vi "Create.vi"(7 "Direction":T1, 8 "error in (no error)":errorcluster, 9 "Custom Config Data":u8[](array[numeric]), 10 "Name":string, 11 "CIFTag in":refnum<class "CIF_Iceoryx_Chn_String.lvclass">) -> (0 "error out":errorcluster, 3 "CIFTag out":refnum<class "CIF_Iceoryx_Chn_String.lvclass">)   [LabVIEW 2021, in "CIF_Iceoryx_Chn_String.lvclass"]
uses:
  CIF_Iceoryx_Chn_String.lvclass
  D:/dev/Packages/CIF_Channels_Core/src/Iceorxy_Channels/CIF_Iceoryx_BB/CIF_Iceoryx_BB.lvclass
  D:/dev/Packages/CIF_Channels_Core/src/CIFChannels/CIFChannels.lvclass
  ChannelCommon/typedef/Direction.ctl
  <vilib>/CIF Foundation/CIF Iceoryx/typedef/Topic Full Names.ctl
  ChannelCommon/typedef/Disconnect Behavior.ctl
  ChannelCommon/typedef/Channel Pattern.ctl
  CIF_Iceoryx_BB/CIF_Iceoryx_BB.lvclass/CIF_Iceoryx_BB.ctl
  ChannelCommon/typedef/Channel State.ctl
  CIFChannels/CIFChannels.lvclass/CIFChannels.ctl
  623fbe6a-c577-42e6-8857-c9eb486a6fdc.vi
  CIF_Iceoryx_BB/Accessors/Write Writer Reference.vi
  CIF_Iceoryx_BB/Accessors/Read Blackboard Reference.vi
  CIF_Iceoryx_BB/Accessors/Write Data Configuration.vi
  CIFChannels/Accessors/Write Pattern.vi
  CIFChannels/Accessors/Write Channel State.vi
  <vilib>/CIF Foundation/CIF Iceoryx/SubVIs/Get Path.vi
  <vilib>/CIF Foundation/CIF Iceoryx/SubVIs/Convert Error.vi
  623fbe6a-c577-42e6-8857-c9eb486a6fdc.vi/3bd89bd1-b605-4b55-aa60-227046f12b11.vi
  <vilib>/CIF Foundation/CIF Iceoryx/SubVIs/Add Error.vi
  <vilib>/CIF Foundation/CIF Iceoryx/Refnum/BB from Refnum.vi
  <vilib>/CIF Foundation/CIF Iceoryx/Refnum/BB Writer to Refnum.vi
  <vilib>/Utility/error.llb/Trim Whitespace.vi
  <vilib>/CIF Foundation/CIF Iceoryx/SubVIs/Add Error Core.vi
  <vilib>/CIF Foundation/CIF Utilities/DataTypes/Utilities/Get Element Info of Variant.vi
  <vilib>/CIF Foundation/CIF Iceoryx/SubVIs/Get Type String.vi
  <vilib>/CIF Foundation/CIF Utilities/DataTypes/Utilities/Get JSON Descriptor of Variant.vi
  <vilib>/CIF Foundation/CIF Iceoryx/SubVIs/Convert Error Core.vi
  CIFChannels/CIFChannels.lvclass
  ChannelCommon/ChannelCommon.lvlib
  <vilib>/CIF Foundation/CIF Iceoryx/Iceoryx.lvlib
  CIF_Iceoryx_BB/CIF_Iceoryx_BB.lvclass
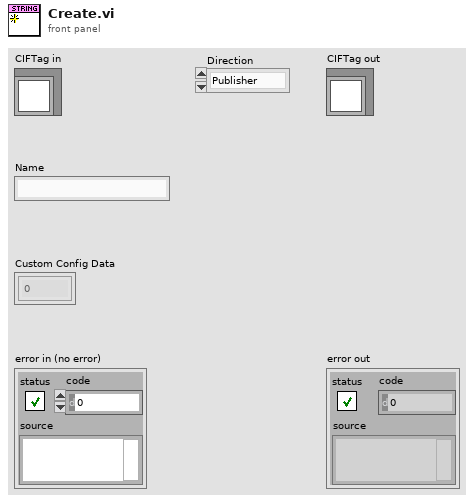
[diagram p1: front panel]
types:
  T1 = typedef "ChannelCommon.lvlib/Direction.ctl" = enum8{"Publisher", "Subscriber"}
  T2 = typedef "Iceoryx.lvlib/Topic Full Names.ctl" = cluster{"BlackBoard":string, "Topic":string, "Type Override":string}
  T3 = typedef "ChannelCommon.lvlib/Disconnect Behavior.ctl" = enum8{"Default value", "Last value", "Error with default"}
  T4 = typedef "ChannelCommon.lvlib/Channel Pattern.ctl" = enum8{"Unknown", "Tag", "FIFO", "MultiFIFO", "BackpressureFIFO"}
  T5 = typedef "ChannelCommon.lvlib/Channel State.ctl" = enum8{"Creating", "Disconnected", "Connecting", "Connected", "Destroyed"}
  T6 = typedef "Iceoryx.lvlib/BB Refnum.ctl" = cluster{"refnum":u64, "BB":enum8{"bb"}}
  T7 = typedef "Iceoryx.lvlib/BB Writer Refnum.ctl" = cluster{"refnum":u64, "BB Writer":enum8{"bb_writer"}}
  T8 = typedef "CIF_Iceoryx_BB.lvclass/Data Configuration.ctl" = cluster{"Element Size":u32, "Element Alignment":u32, "Array":bool, "Type":string}
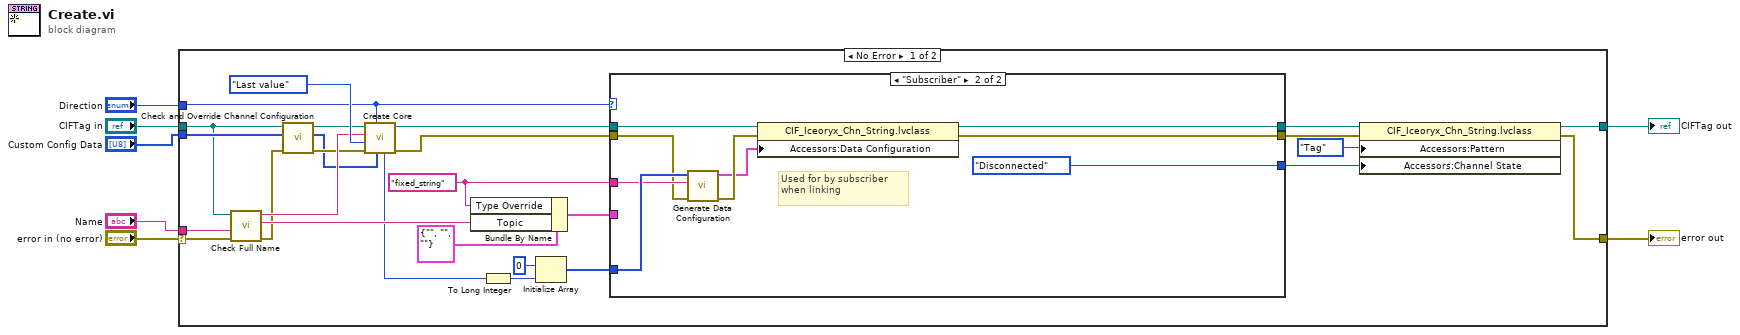
[diagram p0: block diagram]
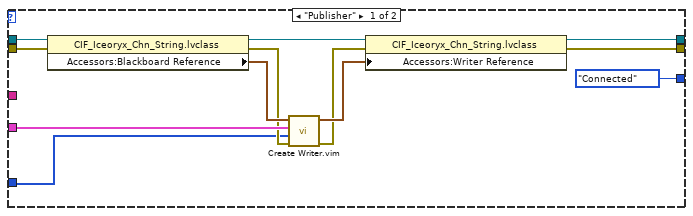
[diagram p2: hidden frame]
diagram:
  n1 = case shown="No Error" "error in (no error)" {
    selector: "error in (no error)" -> [w20 w57]
    tunnel: [w34 w57] -> w1
    tunnel: [w33 w56] -> w2
    tunnel: "CIFTag in" -> [w8 w56]
    tunnel: "Name" -> [w30 _]
    tunnel: "Direction" -> [w23 _]
    tunnel: "Custom Config Data" -> [w21 _]
    frame No Error {
      w9 = "fixed_string" ("Type Override")
      n2 = call "Check Full Name.vi"("error in (no error)"=w20, "Topic Name In"=w30, "CIF_Iceoryx_BB in"=w8) -> ("error out"=w19:errorcluster, "Topic Name out"=w28:string, "Full Name Out"=w29:string)  [unwired: 6 in]
      n3 = call-dynamic "Check and Override Channel Configuration.vi"("error in (no error)"=w19, "Custom Config Data in"=w21, "CIF_CIPC_Chn_String in"=w8) -> ("error out"=w18:errorcluster, "Custom Config Data out"=w17:u8[], "CIF_CIPC_Chn_String out"=w22:refnum<class "CIF_Iceoryx_Chn_String.lvclass">)  [unwired: 6 in]
      n4 = call "Create Core.vi"("Custom Config Data"=w17, "Direction"=w23, "error in (no error)"=w18, "Disconnect Behavior"=Disconnect_Behavior."Last value", "Name"=w29, "CIFChannels in"=w22) -> ("error out"=w11:errorcluster, "CIFChannels out"=w10:refnum<class "CIF_Iceoryx_Chn_String.lvclass">, "Bytes/Msg"=w14:u64)  [unwired: 1 in, 2 out]
      n5 = Bundle By Name(cluster=T2 {"BlackBoard"="", "Topic"="", "Type Override"=""} ("Topic Name"), "Type Override"=w9, "Topic"=w28) -> (w12:T2)
      n6 = To Long Integer(number=w14) -> (32bit integer=w15:i32)
      n7 = Initialize Array(u8 0 ("Buffer Size N (2^N)"), w15) -> (w13:u8[])
      n8 = case shown="\"Subscriber\"" w23 {
        tunnel: [Channel_State."Connected" ("Channel State") Channel_State."Disconnected" ("Channel State")] -> w24
        tunnel: [w45 w54] -> w25
        tunnel: w10 -> [w42 w53]
        tunnel: [w44 w52] -> w26
        tunnel: w13 -> [w35 w49]
        tunnel: w12 -> [w43 _]
        tunnel: w11 -> [w39 w47]
        tunnel: w9 -> [_ w48]
        frame "Publisher" {
          n9 = property class="CIF_Iceoryx_Chn_String.lvclass"(reference=w42, error in=w39) -> (reference out=w40:refnum<class "CIF_Iceoryx_Chn_String.lvclass">, error out=w38:errorcluster, "Accessors:Blackboard Reference"=w41:T6)
          n10 = call "Create Writer.vim"("error in (no error)"=w38, "Data"=w35, "Topic Name"=w43, "BlackBoard Reference"=w41) -> ("error out"=w36:errorcluster, "Writer Reference"=w37:T7)  [unwired: 5 in, 1 out]
          n11 = property class="CIF_Iceoryx_Chn_String.lvclass"(reference=w40, error in=w36, "Accessors:Writer Reference"=w37) -> (reference out=w45:refnum<class "CIF_Iceoryx_Chn_String.lvclass">, error out=w44:errorcluster)
        }
        frame "Subscriber" {
          # "Used for by subscriber when linking"
          n12 = call "Generate Data Configuration.vi"("error in (no error)"=w47, "Cluster or Array String"=w48, "Data"=w49) -> ("error out"=w51:errorcluster, "Data Configuration"=w50:T8)  [unwired: 7 in]
          n13 = property class="CIF_Iceoryx_Chn_String.lvclass"(reference=w53, error in=w51, "Accessors:Data Configuration"=w50) -> (reference out=w54:refnum<class "CIF_Iceoryx_Chn_String.lvclass">, error out=w52:errorcluster)
        }
      }
      n14 = property class="CIF_Iceoryx_Chn_String.lvclass"(reference=w25, error in=w26, "Accessors:Pattern"=Channel_Pattern."Tag" ("Pattern"), "Accessors:Channel State"=w24) -> (reference out=w33:refnum<class "CIF_Iceoryx_Chn_String.lvclass">, error out=w34:errorcluster)
    }
    frame Error {
    }
  }
  "error out" <- w1
  "CIFTag out" <- w2
